vi "Set Max Bar Value.vi"(8 "error in (no error)":errorcluster caption="错误输入（无错误）", 11 "uValue64":u64) -> (0 "error out":errorcluster caption="错误输出", 3 "function return":i32)   [LabVIEW 2017, in "smncsftmt.lvlib"]
doc: "__declspec(dllexport) int SetMaxBarValue(unsigned long long uValue64);"
uses:
  smncsftmt.lvlib
  smncsftmt.dll
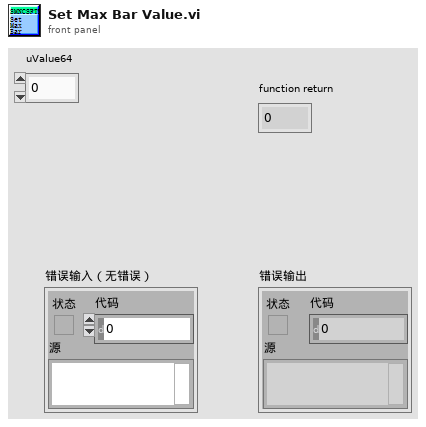
[diagram p1: front panel]
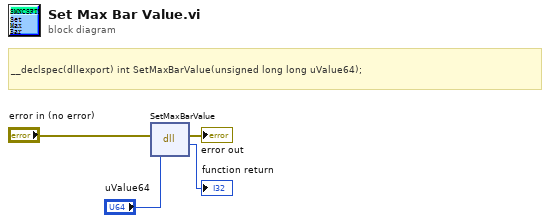
[diagram p0: block diagram]
diagram:
  # "__declspec(dllexport) int SetMaxBarValue(unsigned long long uValue64);"
  n1 = dll-call lib="PTH2oabs CUsersaDesktop\nLABVIEW范例National InstrumentsLabVIEW 2017user.lib\tsmncsftmtsmncsftmt.*" fn="SetMaxBarValue"(error in="error in (no error)", "uValue64"="uValue64") -> (error out=→"error out":errorcluster, "返回类型"=→"function return":i32)  [unwired: 3 in, 1 out]
